vi "temp_path_formation.vi"(8 "error in (no error)":errorcluster) -> (0 "error out":errorcluster, 2 "temp tdms_path":path, 3 "temp txt_path":path)   [LabVIEW 2018]
panel:
  out "temp_txt":string
  out "temp_tdms":string
  out "stripped path":path
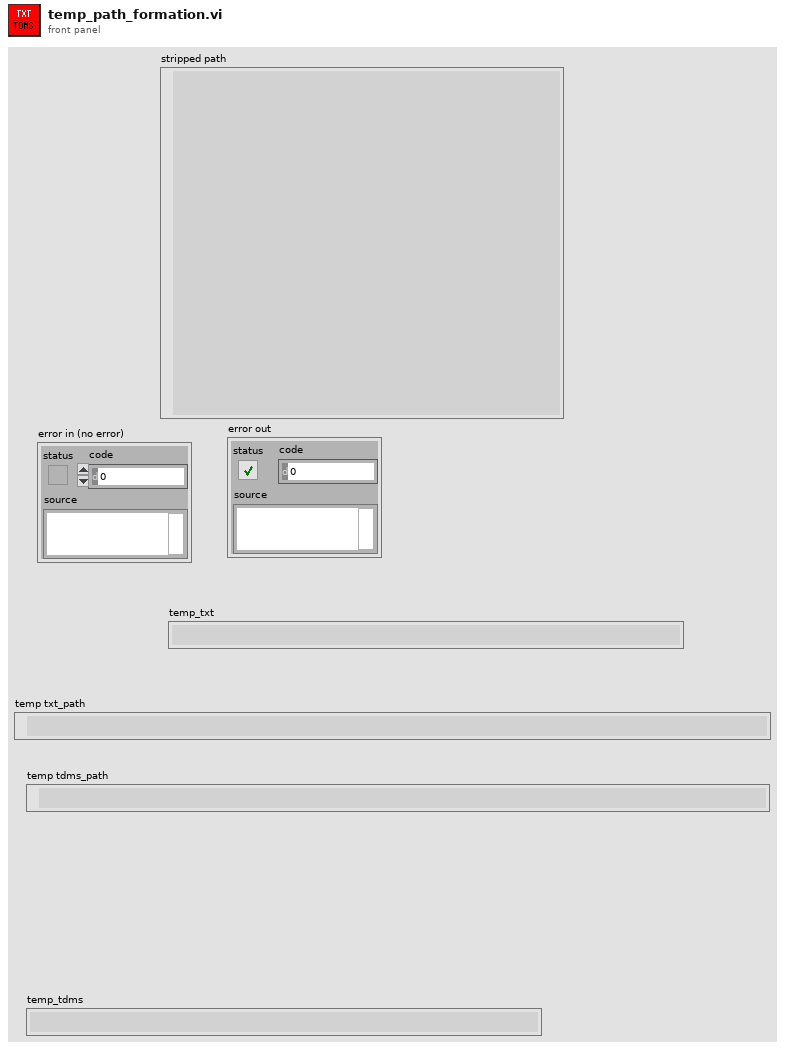
[diagram p1: front panel]
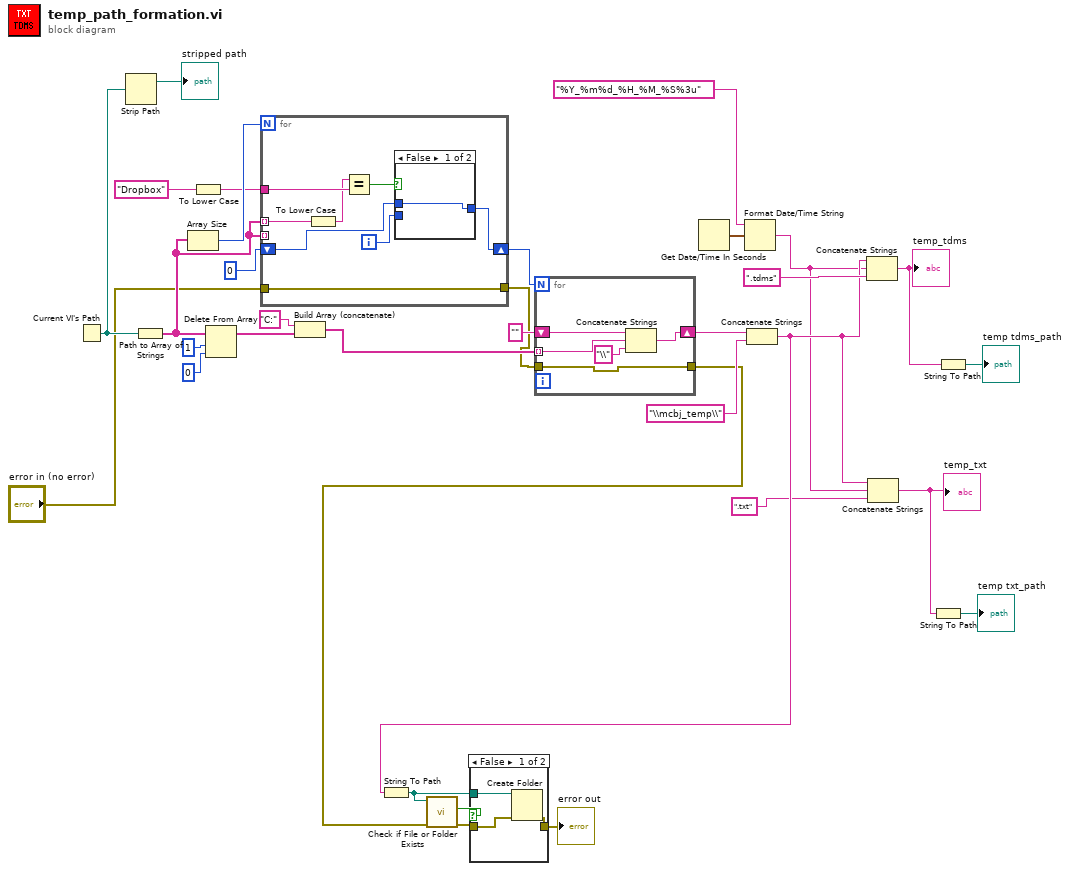
[diagram p0: block diagram]
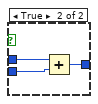
[diagram p3: hidden frame]
diagram:
  n1 = Current VI's Path() -> (path=w31:path)
  n2 = Strip Path(path=w31) -> (stripped path=→"stripped path":path)  [unwired: 1 out]
  n3 = Path to Array of Strings(0:w31) -> (2:w27:string[])  [unwired: 1 out]
  n4 = Array Size(array=w27) -> (size(s)=w30:i32)
  n5 = To Lower Case(string="Dropbox" ("正規表現")) -> (all lower case string=w28:string)
  n6 = Delete From Array(array=w27, length=1, index=0) -> (array with subset deleted=w24:string[])  [unwired: 1 out]
  n7 = for {
    N: w30 -> [_]
    tunnel: w27 -> [w40] mode=indexing
    tunnel: w28 -> [w41]
    tunnel: w27 -> [_] mode=indexing
    shift-right: [w36] -> w19
    shift-left: 0 -> [w35]
    tunnel: "error in (no error)" -> [w34]
    tunnel: [w34] -> w2
    i -> [w37]
    n8 = To Lower Case(string=w40) -> (all lower case string=w39:string)
    n9 = Equal?(x=w39, y=w41) -> (x = y?=w38:bool)
    n10 = case shown="False" w38 {
      tunnel: w37 -> [_ w45]
      tunnel: [w42 w44] -> w36
      tunnel: w35 -> [w42 w43]
      frame False {
      }
      frame True {
        n11 = Add(x=w43, y=w45) -> (x+y=w44:i32)
      }
    }
  }
  n12 = Build Array (concatenate)("C:" ("正規表現"), w24) -> (w22:string[])
  n13 = for {
    N: w19 -> [_]
    tunnel: w22 -> [w49] mode=indexing
    shift-right: [w50] -> w17
    shift-left: "" -> [w48]
    tunnel: w2 -> [w46]
    tunnel: [w46] -> w1
    n14 = Concatenate Strings(w48, w49, "\\" ("string")) -> (w50:string)
  }
  n15 = Get Date/Time In Seconds() -> (seconds since 1Jan1904=w15:timestamp)
  n16 = Format Date/Time String(time format string (%c)="%Y_%m%d_%H_%M_%S%3u" ("時間形式文字列（%c）"), seconds (now)=w15) -> (date/time string=w7:string)  [unwired: 1 in]
  n17 = Concatenate Strings(w17, "\\mcbj_temp\\" ("string")) -> (w8:string)
  n18 = String To Path(string=w8) -> (path=w14:path)
  n19 = call <vilib>:"Check if File or Folder Exists.vi"("error in (no error)"=w1, "path"=w14) -> ("error out"=w12:errorcluster, "file or folder exists?"=w13:bool)  [unwired: 7 in, 1 out]
  n20 = case shown="False" w13 {
    tunnel: w14 -> [w53 _]
    tunnel: w12 -> [w52 w54]
    tunnel: [w51 w54] -> w11
    frame False {
      n21 = Create Folder(path (use dialog)=w53, error in=w52) -> (error out=w51:errorcluster)  [unwired: 1 in, 2 out]
    }
    frame True {
    }
  }
  "error out" <- w11
  n22 = Concatenate Strings(w8, w7, ".tdms" ("string")) -> (w10:string)
  "temp_tdms" <- w10
  n23 = Concatenate Strings(w8, w7, ".txt" ("string")) -> (w4:string)
  "temp_txt" <- w4
  n24 = String To Path(string=w4) -> (path=→"temp txt_path":path)
  n25 = String To Path(string=w10) -> (path=→"temp tdms_path":path)
